vi "Rename Templates.vi"(8 "error in (no error)":errorcluster, 9 "Icon Color":u32(colorbox)=13631442, 10 "VI Refs":refnum<vi>[](array[refnum]), 11 "Subsystem Name":string) -> (0 "error out":errorcluster)   [LabVIEW 2023]
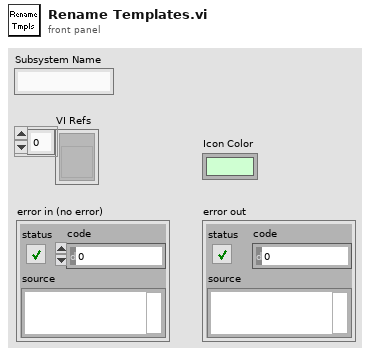
[diagram p1: front panel]
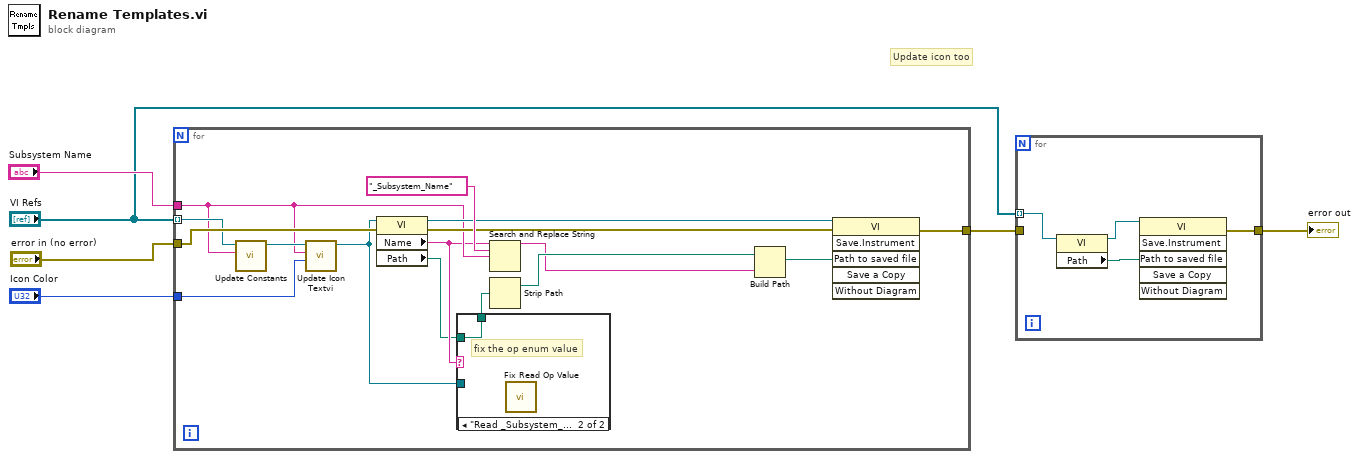
[diagram p0: block diagram]
diagram:
  # "Update icon too"
  n1 = for {
    tunnel: "VI Refs" -> [w14] mode=indexing
    tunnel: "error in (no error)" -> [w17]
    tunnel: "Subsystem Name" -> [w12]
    tunnel: [w16] -> w1
    tunnel: "Icon Color" -> [w11]
    n2 = call <resource>:"Update Constants.vi"("Subsystem Name"=w12, "VI in"=w14) -> ("VI out"=w13:refnum<vi>)  [unwired: 9 in]
    n3 = call <resource>:"Update Icon Textvi.vi"("Icon Color"=w11, "Suubsystem Name"=w12, "vi reference"=w13) -> ("VI Refnum out"=w9:refnum<vi>)  [unwired: 8 in]
    n4 = property class="VI"(reference=w9, error in=w17) -> (reference out=w15:refnum<vi>, error out=w18:errorcluster, "Name"=w10:string, "Path"=w8:path)
    n5 = case shown="\"Read _Subsystem_Name Operation.vi\"" w10 {
      tunnel: w9 -> [_ _]
      tunnel: w8 -> [w23 w24]
      tunnel: [w23 w24] -> w7
      frame Default {
      }
      frame "Read _Subsystem_Name Operation.vi" {
        # "fix the op enum value"
        n6 = call <resource>:"Fix Read Op Value.vi"() -> ()  [unwired: 11 in, 1 out]
      }
    }
    n7 = Search and Replace String(input string=w10, search string="_Subsystem_Name", replace string=w12) -> (result string=w20:string)  [unwired: 5 in, 3 out]
    n8 = Strip Path(path=w7) -> (stripped path=w21:path)  [unwired: 1 out]
    n9 = Build Path(base path=w21, name or relative path=w20) -> (appended path=w19:path)
    n10 = invoke class="VI" method="Save.Instrument"(reference=w15, error in=w18, "Path to saved file"=w19) -> (error out=w16:errorcluster)  [unwired: 3 in, 5 out]
  }
  n11 = for {
    tunnel: [w28] -> w3
    tunnel: "VI Refs" -> [w26] mode=indexing
    tunnel: w1 -> [_]
    n12 = property class="VI"(reference=w26) -> (reference out=w25:refnum<vi>, "Path"=w27:path)  [unwired: 1 in, 1 out]
    n13 = invoke class="VI" method="Save.Instrument"(reference=w25, "Path to saved file"=w27) -> (error out=w28:errorcluster)  [unwired: 4 in, 5 out]
  }
  "error out" <- w3
